vi "test modern errors.vi"(8 "error in (no error)":errorcluster) -> (0 "error out":errorcluster, 3 "body":string)   [LabVIEW 2020, in "MCP Server tests.lvlib"]
doc: "Modern requests that cannot be served: a version that is not a modern one gives HTTP 400 with error -32022 Unsupported protocol version and data.supported (all versions) and data.requested; missing clientCapabilities gives 400 with -32602; a method the modern era does not have (also ping) gives HTTP 404 with -32601; resources/read of an unknown uri gives -32602 instead of the legacy -32002. The requests are sent with the LabVIEW HTTP Client directly."
uses:
  MCP Server tests.lvlib
  1c452fb1-ba73-480b-9343-900331c420b7.vi
  8f5dcdb6-db46-4e8a-aade-ac0ff40d6022.vi
  <vilib>/JDP Science/JSONtext/Next JSON Value.vi
  <vilib>/JDP Science/JSONtext/String Subset.vi
  <vilib>/JDP Science/JSONtext/Parsing/Advance past next JSON Value (inlined COPY).vi
  <vilib>/JDP Science/JSONtext/Parsing/Advance past whitespace.vi
  <vilib>/JDP Science/JSONtext/Parsing/Advance past String.vi
  <vilib>/JDP Science/JSONtext/Parsing/Advance past Number.vi
  <vilib>/JDP Science/JSONtext/Parsing/Advance past Line Ending.vi
  <vilib>/JDP Science/JSONtext/Parsing/Parse Full Path or Item Name.vi
  <vilib>/JDP Science/JSONtext/Parsing/Advance past Array.vi
  <vilib>/JDP Science/JSONtext/Parsing/Advance past Object.vi
  <vilib>/JDP Science/JSONtext/support/Error Cluster From Code.vi
  <vilib>/JDP Science/JSONtext/Offset/Find Item Locations by Path.vi
  <vilib>/JDP Science/JSONtext/JSON text to Variant.vi
  <vilib>/JDP Science/JSONtext/LVClass Serializer/JSONtext LVClass Serializer.lvclass
  <vilib>/addons/_JKI Toolkits/Caraya/classes/Test/Test.lvclass
  <vilib>/JDP Science/JSONtext/JSONtext.lvlib
  <vilib>/addons/_JKI Toolkits/Caraya/classes/Assert/Assert.lvclass
panel:
  out "lookup error":errorcluster
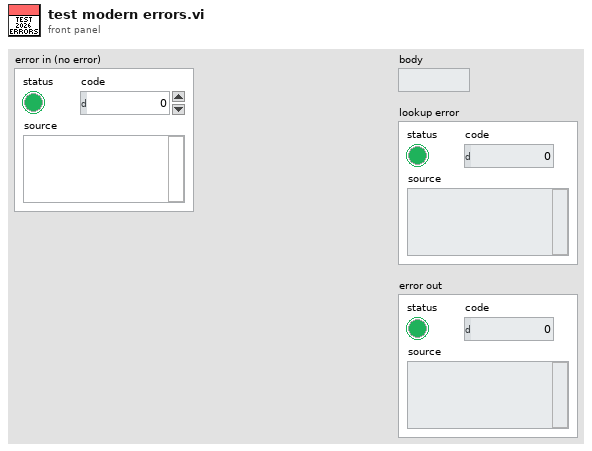
[diagram p1: front panel]
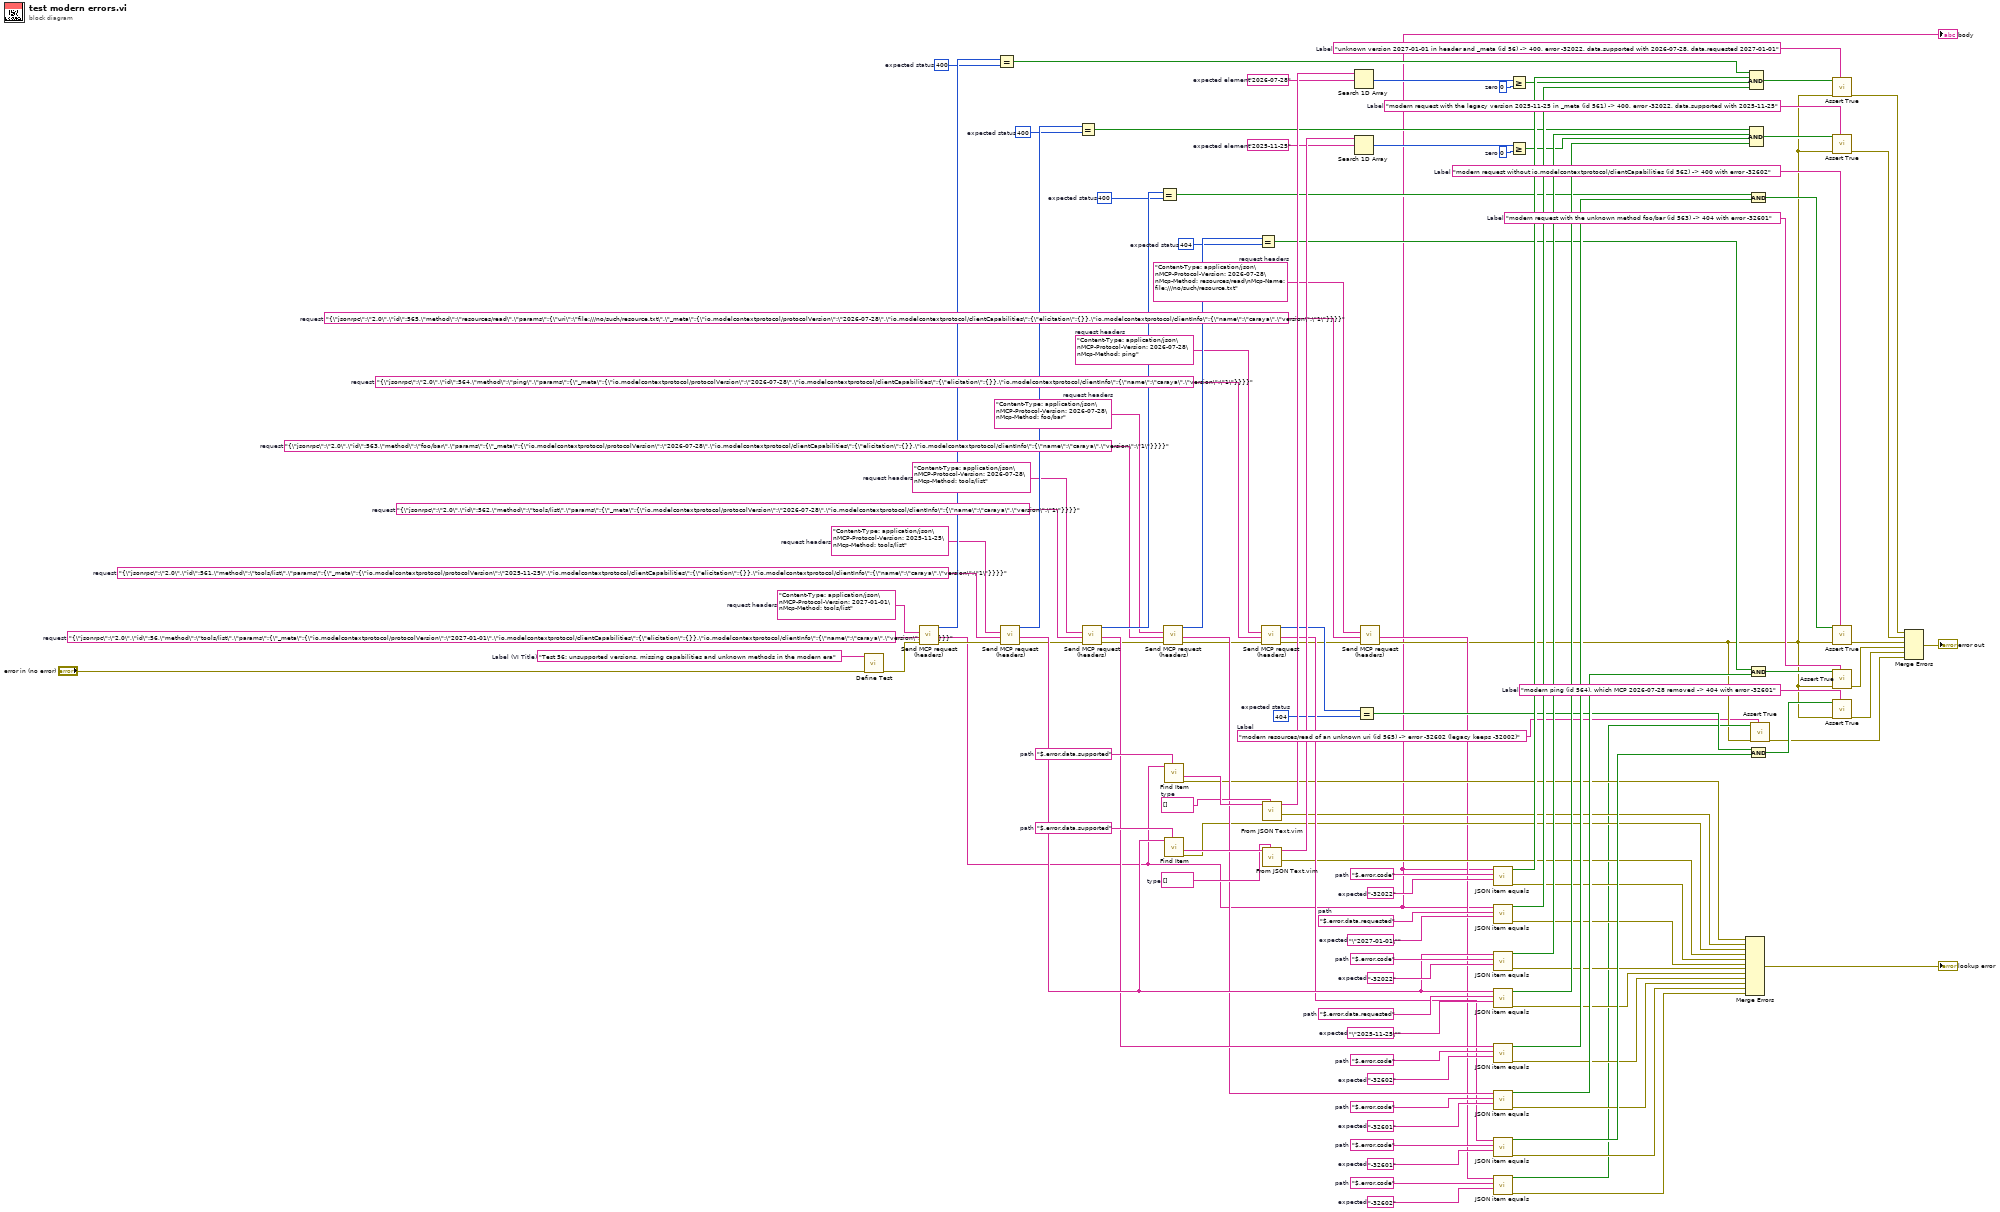
[diagram p0: block diagram]
diagram:
  w40 = "Content-Type: application/json\nMCP-Protocol-Version: 2026-07-28\nMcp-Method: resources/read\nMcp-Name: file:///no/such/resource.txt"  # request headers
  w50 = "Content-Type: application/json\nMCP-Protocol-Version: 2026-07-28\nMcp-Method: ping"  # request headers
  w60 = "Content-Type: application/json\nMCP-Protocol-Version: 2026-07-28\nMcp-Method: foo/bar"  # request headers
  w70 = "Content-Type: application/json\nMCP-Protocol-Version: 2026-07-28\nMcp-Method: tools/list"  # request headers
  w91 = "Content-Type: application/json\nMCP-Protocol-Version: 2025-11-25\nMcp-Method: tools/list"  # request headers
  w111 = "Content-Type: application/json\nMCP-Protocol-Version: 2027-01-01\nMcp-Method: tools/list"  # request headers
  w10 = "modern resources/read of an unknown uri (id 565) -> error -32602 (legacy keeps -32002)"  # Label
  w13 = "modern ping (id 564), which MCP 2026-07-28 removed -> 404 with error -32601"  # Label
  w15 = "modern request with the unknown method foo/bar (id 563) -> 404 with error -32601"  # Label
  w17 = "modern request without io.modelcontextprotocol/clientCapabilities (id 562) -> 400 with error -32602"  # Label
  w19 = "modern request with the legacy version 2025-11-25 in _meta (id 561) -> 400, error -32022, data.supported with 2025-11-25"  # Label
  w21 = "unknown version 2027-01-01 in header and _meta (id 56) -> 400, error -32022, data.supported with 2026-07-28, data.requested 2027-01-01"  # Label
  w24 = "-32602"  # expected
  w25 = "$.error.code"  # path
  w45 = "-32601"  # expected
  w46 = "$.error.code"  # path
  w43 = 404  # expected status
  w55 = "-32601"  # expected
  w56 = "$.error.code"  # path
  w53 = 404  # expected status
  w65 = "-32602"  # expected
  w66 = "$.error.code"  # path
  w63 = 400  # expected status
  w81 = "\"2025-11-25\""  # expected
  w82 = "$.error.data.requested"  # path
  w75 = 0  # zero
  w77 = "2025-11-25"  # expected element
  w84 = "-32022"  # expected
  w85 = "$.error.code"  # path
  w79 = 400  # expected status
  w102 = "\"2027-01-01\""  # expected
  w103 = "$.error.data.requested"  # path
  w96 = 0  # zero
  w98 = "2026-07-28"  # expected element
  w104 = "-32022"  # expected
  w105 = "$.error.code"  # path
  w100 = 400  # expected status
  w86 = string[] []  # type
  w88 = "$.error.data.supported"  # path
  w106 = string[] []  # type
  w108 = "$.error.data.supported"  # path
  w39 = "{\"jsonrpc\":\"2.0\",\"id\":565,\"method\":\"resources/read\",\"params\":{\"uri\":\"file:///no/such/resource.txt\",\"_meta\":{\"io.modelcontextprotocol/protocolVersion\":\"2026-07-28\",\"io.modelcontextprotocol/clientCapabilities\":{\"elicitation\":{}},\"io.modelcontextprotocol/clientInfo\":{\"name\":\"caraya\",\"version\":\"1\"}}}}"  # request
  w49 = "{\"jsonrpc\":\"2.0\",\"id\":564,\"method\":\"ping\",\"params\":{\"_meta\":{\"io.modelcontextprotocol/protocolVersion\":\"2026-07-28\",\"io.modelcontextprotocol/clientCapabilities\":{\"elicitation\":{}},\"io.modelcontextprotocol/clientInfo\":{\"name\":\"caraya\",\"version\":\"1\"}}}}"  # request
  w59 = "{\"jsonrpc\":\"2.0\",\"id\":563,\"method\":\"foo/bar\",\"params\":{\"_meta\":{\"io.modelcontextprotocol/protocolVersion\":\"2026-07-28\",\"io.modelcontextprotocol/clientCapabilities\":{\"elicitation\":{}},\"io.modelcontextprotocol/clientInfo\":{\"name\":\"caraya\",\"version\":\"1\"}}}}"  # request
  w69 = "{\"jsonrpc\":\"2.0\",\"id\":562,\"method\":\"tools/list\",\"params\":{\"_meta\":{\"io.modelcontextprotocol/protocolVersion\":\"2026-07-28\",\"io.modelcontextprotocol/clientInfo\":{\"name\":\"caraya\",\"version\":\"1\"}}}}"  # request
  w90 = "{\"jsonrpc\":\"2.0\",\"id\":561,\"method\":\"tools/list\",\"params\":{\"_meta\":{\"io.modelcontextprotocol/protocolVersion\":\"2025-11-25\",\"io.modelcontextprotocol/clientCapabilities\":{\"elicitation\":{}},\"io.modelcontextprotocol/clientInfo\":{\"name\":\"caraya\",\"version\":\"1\"}}}}"  # request
  w110 = "{\"jsonrpc\":\"2.0\",\"id\":56,\"method\":\"tools/list\",\"params\":{\"_meta\":{\"io.modelcontextprotocol/protocolVersion\":\"2027-01-01\",\"io.modelcontextprotocol/clientCapabilities\":{\"elicitation\":{}},\"io.modelcontextprotocol/clientInfo\":{\"name\":\"caraya\",\"version\":\"1\"}}}}"  # request
  w113 = "Test 56: unsupported versions, missing capabilities and unknown methods in the modern era"  # Label (VI Title)
  n1 = call <vilib>:"Define Test.vi"("error in (no error)"="error in (no error)", "Label (VI Title)"=w113) -> ("error out"=w109:errorcluster)  [unwired: 8 in, 1 out]
  n2 = call "Send MCP request (headers).vi"("error in (no error)"=w109, "request"=w110, "request headers"=w111) -> ("error out"=w89:errorcluster, "response"=w3:string, "status code"=w101:i32)  [unwired: 5 in, 1 out]
  "body" <- w3
  n3 = Equal?(x=w101, y=w100) -> (x = y?=w95:bool)
  n4 = call "Send MCP request (headers).vi"("error in (no error)"=w89, "request"=w90, "request headers"=w91) -> ("error out"=w68:errorcluster, "response"=w83:string, "status code"=w80:i32)  [unwired: 5 in, 1 out]
  n5 = Equal?(x=w80, y=w79) -> (x = y?=w74:bool)
  n6 = call "Send MCP request (headers).vi"("error in (no error)"=w68, "request"=w69, "request headers"=w70) -> ("error out"=w58:errorcluster, "response"=w67:string, "status code"=w64:i32)  [unwired: 5 in, 1 out]
  n7 = Equal?(x=w64, y=w63) -> (x = y?=w62:bool)
  n8 = call "Send MCP request (headers).vi"("error in (no error)"=w58, "request"=w59, "request headers"=w60) -> ("error out"=w48:errorcluster, "response"=w57:string, "status code"=w54:i32)  [unwired: 5 in, 1 out]
  n9 = call <vilib>:"Find Item.vi"("$Path or Item Name"=w108, "JSON"=w3) -> ("error out"=w37:errorcluster, "<JSON>"=w107:string)  [unwired: 6 in, 2 out]
  n10 = call <vilib>:"Find Item.vi"("$Path or Item Name"=w88, "JSON"=w83) -> ("error out"=w35:errorcluster, "<JSON>"=w87:string)  [unwired: 6 in, 2 out]
  n11 = Equal?(x=w54, y=w53) -> (x = y?=w52:bool)
  n12 = call "Send MCP request (headers).vi"("error in (no error)"=w48, "request"=w49, "request headers"=w50) -> ("error out"=w38:errorcluster, "response"=w47:string, "status code"=w44:i32)  [unwired: 5 in, 1 out]
  n13 = call "From JSON Text.vim"("Data Type and Default Value"=w106, "JSON"=w107) -> ("error out"=w36:errorcluster, "Data out"=w99:string[])  [unwired: 8 in]
  n14 = call "From JSON Text.vim"("Data Type and Default Value"=w86, "JSON"=w87) -> ("error out"=w34:errorcluster, "Data out"=w78:string[])  [unwired: 8 in]
  n15 = Search 1D Array(1D array=w99, element=w98) -> (index of element=w97:i32)  [unwired: 1 in]
  n16 = Search 1D Array(1D array=w78, element=w77) -> (index of element=w76:i32)  [unwired: 1 in]
  n17 = Equal?(x=w44, y=w43) -> (x = y?=w42:bool)
  n18 = call "Send MCP request (headers).vi"("error in (no error)"=w38, "request"=w39, "request headers"=w40) -> ("error out"=w11:errorcluster, "response"=w26:string)  [unwired: 5 in, 2 out]
  n19 = call "JSON item equals.vi"("expected"=w104, "path"=w105, "JSON"=w3) -> ("error out"=w33:errorcluster, "equal?"=w94:bool)  [unwired: 6 in, 1 out]
  n20 = call "JSON item equals.vi"("expected"=w102, "path"=w103, "JSON"=w3) -> ("error out"=w32:errorcluster, "equal?"=w92:bool)  [unwired: 6 in, 1 out]
  n21 = call "JSON item equals.vi"("expected"=w84, "path"=w85, "JSON"=w83) -> ("error out"=w31:errorcluster, "equal?"=w73:bool)  [unwired: 6 in, 1 out]
  n22 = call "JSON item equals.vi"("expected"=w81, "path"=w82, "JSON"=w83) -> ("error out"=w30:errorcluster, "equal?"=w71:bool)  [unwired: 6 in, 1 out]
  n23 = call "JSON item equals.vi"("expected"=w65, "path"=w66, "JSON"=w67) -> ("error out"=w29:errorcluster, "equal?"=w61:bool)  [unwired: 6 in, 1 out]
  n24 = call "JSON item equals.vi"("expected"=w55, "path"=w56, "JSON"=w57) -> ("error out"=w28:errorcluster, "equal?"=w51:bool)  [unwired: 6 in, 1 out]
  n25 = call "JSON item equals.vi"("expected"=w45, "path"=w46, "JSON"=w47) -> ("error out"=w27:errorcluster, "equal?"=w41:bool)  [unwired: 6 in, 1 out]
  n26 = call "JSON item equals.vi"("expected"=w24, "path"=w25, "JSON"=w26) -> ("error out"=w23:errorcluster, "equal?"=w12:bool)  [unwired: 6 in, 1 out]
  n27 = Greater Or Equal?(x=w97, y=w96) -> (x >= y?=w93:bool)
  n28 = Greater Or Equal?(x=w76, y=w75) -> (x >= y?=w72:bool)
  n29 = Merge Errors(w37, w36, w35, w34, w33, w32, w31, w30, w29, w28, w27, w23) -> (→"lookup error":errorcluster)
  n30 = Compound Arithmetic op=AND(w95, w94, w93, w92) -> (w22:bool)
  n31 = Compound Arithmetic op=AND(w74, w73, w72, w71) -> (w20:bool)
  n32 = call <vilib>:"Assert True.vi"("Label"=w10, "error in (no error)"=w11, "True?"=w12) -> ("error out"=w4:errorcluster)  [unwired: 7 in, 1 out]
  n33 = Compound Arithmetic op=AND(w62, w61) -> (w18:bool)
  n34 = Compound Arithmetic op=AND(w52, w51) -> (w16:bool)
  n35 = Compound Arithmetic op=AND(w42, w41) -> (w14:bool)
  n36 = call <vilib>:"Assert True.vi"("Label"=w21, "error in (no error)"=w11, "True?"=w22) -> ("error out"=w9:errorcluster)  [unwired: 7 in, 1 out]
  n37 = call <vilib>:"Assert True.vi"("Label"=w19, "error in (no error)"=w11, "True?"=w20) -> ("error out"=w8:errorcluster)  [unwired: 7 in, 1 out]
  n38 = call <vilib>:"Assert True.vi"("Label"=w17, "error in (no error)"=w11, "True?"=w18) -> ("error out"=w7:errorcluster)  [unwired: 7 in, 1 out]
  n39 = call <vilib>:"Assert True.vi"("Label"=w15, "error in (no error)"=w11, "True?"=w16) -> ("error out"=w6:errorcluster)  [unwired: 7 in, 1 out]
  n40 = call <vilib>:"Assert True.vi"("Label"=w13, "error in (no error)"=w11, "True?"=w14) -> ("error out"=w5:errorcluster)  [unwired: 7 in, 1 out]
  n41 = Merge Errors(w9, w8, w7, w6, w5, w4) -> (→"error out":errorcluster)
